vi "resizeDialog.vi"(2 "error in (no error)":errorcluster, 3 "caller VI ref":refnum<vi>, 4 "Cancel button refnum":refnum<vi>, 5 "launch time?":bool, 6 "OK button refnum":refnum<vi>, 7 "Pict Refnum":refnum<vi>, 8 "Default env string refnum":refnum<vi>, 9 "Do show again checkbox refnum":refnum<vi>, 10 "invoke it string efnum":refnum<vi>, 11 "Pict Refnum":refnum<vi>) -> (0 "error out":errorcluster)   [LabVIEW 2023]
panel:
  in  "Cancel":string="Cancel"
  in  "Apply":string="Apply"
  in  "cancel button text":string="Exit"
  in  "OK button text":string="Start LabVIEW"
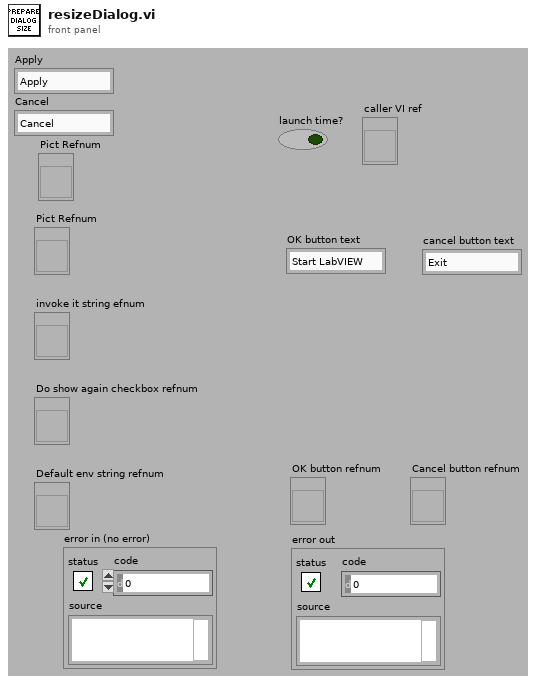
[diagram p1: front panel]
types:
  T1 = enum32{"Invalid", "Standard", "Closed", "Hidden", "Minimized", "Maximized"}
  T2 = typedef "LVRectTypeDef.ctl" = cluster{"Left":i16, "Top":i16, "Right":i16, "Bottom":i16}
  T3 = typedef "LVPointTypeDef.ctl" = cluster{"Horizontal":i16, "Vertical":i16}
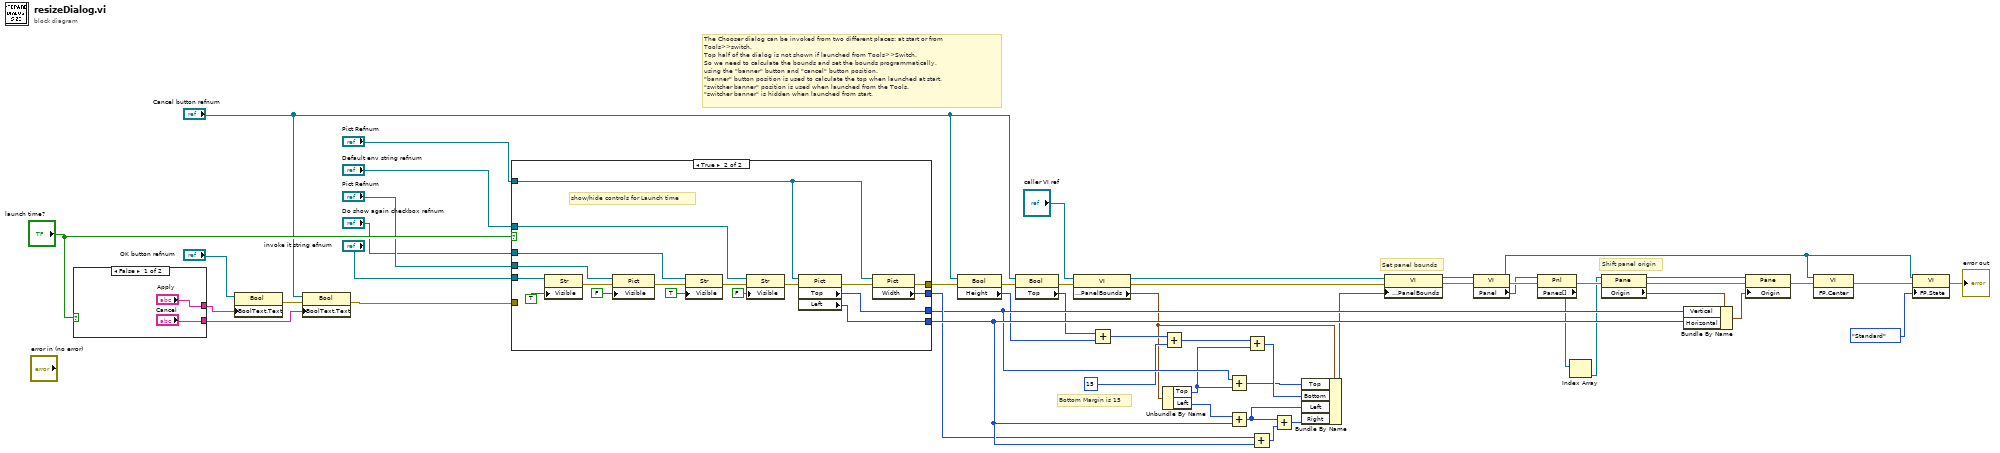
[diagram p0: block diagram]
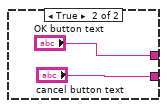
[diagram p2: hidden frame]
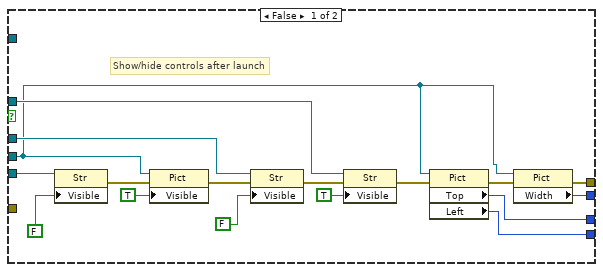
[diagram p3: hidden frame]
diagram:
  # "The Chooser dialog can be invoked from two different places: at start or from Tools>>switch. \nTop half of the dialog is not shown if launched from Tools>>Switch.\nSo we need to calculate the bounds and set the bounds programmatically, \nusing the \"banner\" button and \"cancel\" button position.\n\"banner\" button position is used to calculate the top when launched at start. \n\"switcher banner\" position is used when launched from the Tools.\n\"switcher banner\" is hidden when launched from start."
  # "Shift panel origin"
  # "Set panel bounds"
  # "Bottom Margin is 15"
  n1 = case shown="False" "launch time?" {
    tunnel: ["Cancel" "cancel button text"] -> w7
    tunnel: ["Apply" "OK button text"] -> w8
    frame False {
    }
    frame True {
    }
  }
  n2 = property on="Property Node" class="Bool"(reference="OK button refnum", "BoolText.Text"=w8) -> (error out=w9:errorcluster)  [unwired: 1 in, 1 out]
  n3 = property on="Property Node" class="Bool"(reference="Cancel button refnum", error in=w9, "BoolText.Text"=w7) -> (error out=w11:errorcluster)  [unwired: 1 out]
  n4 = case shown="True" "launch time?" {
    tunnel: [w72 w90] -> w38
    tunnel: [w68 w86] -> w33
    tunnel: [w71 w89] -> w47
    tunnel: [w69 w88] -> w43
    tunnel: "Pict Refnum" -> [w64 w82]
    tunnel: "Do show again checkbox refnum" -> [w66 w81]
    tunnel: "Default env string refnum" -> [w65 w83]
    tunnel: "invoke it string efnum" -> [w63 w85]
    tunnel: "Pict Refnum" -> [_ w84]
    tunnel: w11 -> [_ _]
    frame False {
      # "Show/hide controls after launch"
      n5 = property on="Property Node" class="Str"(reference=w63, "Visible"=FALSE) -> (error out=w60:errorcluster)  [unwired: 1 in, 1 out]
      n6 = property on="Property Node" class="Pict"(reference=w64, error in=w60, "Visible"=TRUE) -> (error out=w59:errorcluster)  [unwired: 1 out]
      n7 = property on="Property Node" class="Str"(reference=w66, error in=w59, "Visible"=FALSE) -> (error out=w57:errorcluster)  [unwired: 1 out]
      n8 = property on="Property Node" class="Str"(reference=w65, error in=w57, "Visible"=TRUE) -> (error out=w67:errorcluster)  [unwired: 1 out]
      n9 = property on="Property Node" class="Pict"(reference=w64, error in=w67) -> (error out=w70:errorcluster, "Top"=w72:i32, "Left"=w71:i32)  [unwired: 1 out]
      n10 = property on="Property Node" class="Pict"(reference=w64, error in=w70) -> (error out=w68:errorcluster, "Width"=w69:u32)  [unwired: 1 out]
    }
    frame True {
      # "show/hide controls for Launch time"
      n11 = property on="Property Node" class="Str"(reference=w85, "Visible"=TRUE) -> (error out=w78:errorcluster)  [unwired: 1 in, 1 out]
      n12 = property on="Property Node" class="Pict"(reference=w82, error in=w78, "Visible"=FALSE) -> (error out=w76:errorcluster)  [unwired: 1 out]
      n13 = property on="Property Node" class="Str"(reference=w81, error in=w76, "Visible"=TRUE) -> (error out=w74:errorcluster)  [unwired: 1 out]
      n14 = property on="Property Node" class="Str"(reference=w83, error in=w74, "Visible"=FALSE) -> (error out=w80:errorcluster)  [unwired: 1 out]
      n15 = property on="Property Node" class="Pict"(reference=w84, error in=w80) -> (error out=w87:errorcluster, "Top"=w90:i32, "Left"=w89:i32)  [unwired: 1 out]
      n16 = property on="Property Node" class="Pict"(reference=w84, error in=w87) -> (error out=w86:errorcluster, "Width"=w88:u32)  [unwired: 1 out]
    }
  }
  n17 = property on="Property Node" class="Bool"(reference="Cancel button refnum", error in=w33) -> (error out=w32:errorcluster, "Height"=w35:u32)  [unwired: 1 out]
  n18 = property on="Property Node" class="Bool"(reference="Cancel button refnum", error in=w32) -> (error out=w50:errorcluster, "Top"=w34:i32)  [unwired: 1 out]
  n19 = property class="VI"(reference="caller VI ref", error in=w50) -> (reference out=w13:refnum<vi>, error out=w3:errorcluster, "Front Panel.PanelBounds"=w29:T2)
  n20 = Add(x=w34, y=w35) -> (x+y=w36:u32)
  n21 = Unbundle By Name(w29) -> ("Top"=w37:i16, "Left"=w42:i16)
  n22 = Add(x=w36, y=u32 15) -> (x+y=w40:u32)
  n23 = Add(x=w38, y=w37) -> (x+y=w39:i32)
  n24 = Add(x=w42, y=w47) -> (x+y=w44:i32)
  n25 = Add(x=w40, y=w37) -> (x+y=w41:u32)
  n26 = Add(x=w43, y=w47) -> (x+y=w45:u32)
  n27 = Add(x=w44, y=w45) -> (x+y=w46:u32)
  n28 = Bundle By Name(cluster=w29, "Top"=w39, "Bottom"=w41, "Left"=w44, "Right"=w46) -> (w28:T2)
  n29 = property class="VI"(reference=w13, error in=w3, "Front Panel.PanelBounds"=w28) -> (reference out=w14:refnum<vi>, error out=w2:errorcluster)
  n30 = property class="VI"(reference=w14, error in=w2) -> (reference out=w1:refnum<vi>, error out=w48:errorcluster, "Panel"=w27:refnum<vi>)
  n31 = property class="Pnl"(reference=w27, error in=w48) -> (error out=w49:errorcluster, "Panes[]"=w22:refnum<vi>[])  [unwired: 1 out]
  n32 = Index Array(array=w22) -> (element=w31:refnum<vi>)  [unwired: 1 in]
  n33 = property class="Pane"(reference=w31, error in=w49) -> (reference out=w26:refnum<vi>, error out=w23:errorcluster, "Origin"=w24:T3)
  n34 = Bundle By Name(cluster=w24, "Vertical"=w38, "Horizontal"=w47) -> (w25:T3)
  n35 = property class="Pane"(reference=w26, error in=w23, "Origin"=w25) -> (error out=w5:errorcluster)  [unwired: 1 out]
  n36 = invoke class="VI" method="FP.Center"(reference=w1, error in=w5) -> (error out=w4:errorcluster)  [unwired: 1 in, 2 out]
  n37 = property on="Property Node" class="VI"(reference=w1, error in=w4, "FP.State"=T1."Standard" ("Front Panel Window:State")) -> (error out=→"error out":errorcluster)  [unwired: 1 out]
